vi "CE - PSD Marker Type.vi"(8 "error in (no error)":errorcluster, 11 "SA Measurement in":refnum<class "SA Measurement.lvclass">) -> (0 "error out":errorcluster, 3 "SA Measurement out":refnum<class "SA Measurement.lvclass">)   [LabVIEW 2023, in "Spectrum Analyzer.lvlib" / "SA Measurement.lvclass"]
uses:
  SA Measurement.lvclass
  SA Measurement.lvclass/SA Measurement.ctl
  Keysight 9020A/Keysight 9020A.lvclass
  TYPE DEFINITION/TYPE Y-axis Unit.ctl
  Spectrum Analyzer.lvlib
  TYPE DEFINITION/TYPE Start and Stop Frequency.ctl
  TYPE DEFINITION/TYPE Center and Span Frequency.ctl
  TYPE DEFINITION/TYPE Reference Level and Atten Param.ctl
  TYPE DEFINITION/TYPE Display Trace Mode Select.ctl
  TYPE DEFINITION/TYPE Detect Mode Select.ctl
  TYPE DEFINITION/TYPE Average Mode Select.ctl
  TYPE DEFINITION/SA Measurement Class/TYPE CE PSD Setting Parameter.ctl
  D:/Project/IST013_CE Conduction Measurement/IST013-CE-Condcuted-Measurement/src/Spectrum Analyzer/Interface_Spectrum/Interface_Spectrum.lvclass
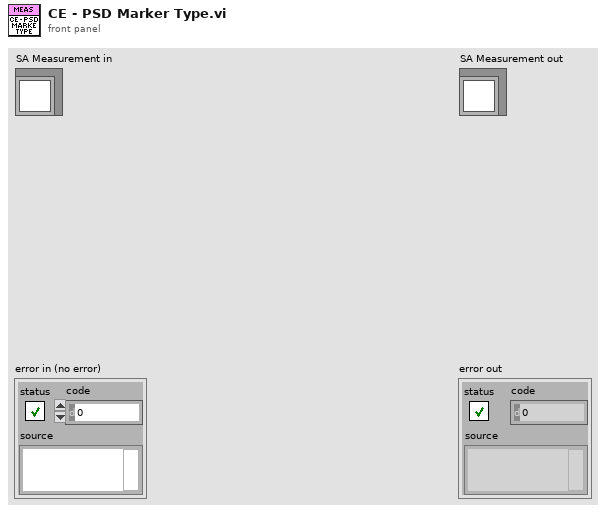
[diagram p1: front panel]
types:
  T1 = typedef "Spectrum Analyzer.lvlib/TYPE CE PSD Setting Parameter.ctl" = cluster{"Y-axis Unit":T2, "Start/Stop Frequency(Hz)":T3, "Center and Span Frequency(Hz)":T4, "PSD Type":enum16{"Marker", "Trace"}, "Ref and Atten":T5, "External Loss":dbl, "RBW/VBW(Hz)":cluster{"RBW":dbl, "VBW":dbl}, "Sweep Point":u32, "Sweep Time(s)":cluster{"Time":dbl, "Auto?":bool}, "Trace and Detect":cluster{"Trace Mode":T6, "Detector Type":T7, "Detect Auto?":bool}[], "Average Mode":T8, "Avg/Hold Number":u32}
  T2 = typedef "Spectrum Analyzer.lvlib/TYPE Y-axis Unit.ctl" = enum16{"dBm", "dBmV", "dBuV", "dBpW", "Volt", "Ampere", "Watt"}
  T3 = typedef "Spectrum Analyzer.lvlib/TYPE Start and Stop Frequency.ctl" = cluster{"Start":dbl, "Stop":dbl}
  T4 = typedef "Spectrum Analyzer.lvlib/TYPE Center and Span Frequency.ctl" = cluster{"Center":dbl, "Span":dbl}
  T5 = typedef "Spectrum Analyzer.lvlib/TYPE Reference Level and Atten Param.ctl" = cluster{"Reference Level":dbl, "Atten":i32, "Atten Auto?":bool, "Reference Level Offset":dbl}
  T6 = typedef "Spectrum Analyzer.lvlib/TYPE Display Trace Mode Select.ctl" = enum16{"Clear Write", "Max Hold", "Min Hold", "Average", "View"}
  T7 = typedef "Spectrum Analyzer.lvlib/TYPE Detect Mode Select.ctl" = enum16{"Det Auto (Normal)", "Auto Peak", "Positive Peak", "Negative Peak", "Sample", "RMS", "Average", "Quasipeak", "CISPR Average", "RMS Average"}
  T8 = typedef "Spectrum Analyzer.lvlib/TYPE Average Mode Select.ctl" = enum16{"Linear(Voltage Avg)", "Video(Log)", "Power"}
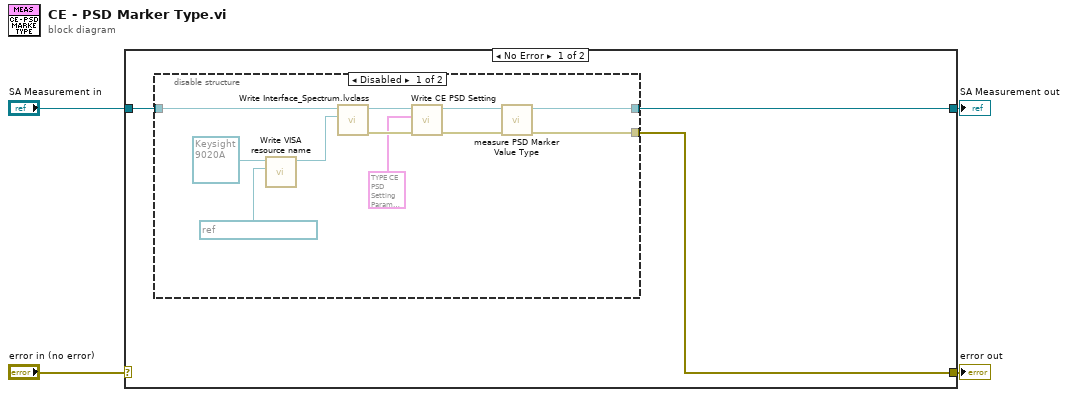
[diagram p0: block diagram]
diagram:
  n1 = case shown="No Error" "error in (no error)" {
    selector: "error in (no error)" -> [_ w20]
    tunnel: [w5 w20] -> w3
    tunnel: [w6 w19] -> w1
    tunnel: "SA Measurement in" -> [w7 w19]
    frame No Error {
      n2 = disable-structure shown="Disabled" {
        disable-tunnel: w7 -> [w16 _]
        disable-tunnel: [w10 _] -> w6
        disable-tunnel: [w8 _] -> w5
        frame Disabled {
          n3 = call "Write VISA resource name.vi"("VISA resource name"=refnum<visa-resource-name> "GPIB0::18::INSTR", "Keysight 9020A in"=refnum<class "Keysight 9020A.lvclass"> refnum ("Spectrum Analyzer.lvlib:Keysight 9020A.lvclass")) -> ("Keysight 9020A out"=w15:refnum<class "Keysight 9020A.lvclass">)  [unwired: 8 in, 1 out]
          n4 = call "Write Interface_Spectrum.lvclass.vi"("Interface_Spectrum.lvclass"=w15, "SA Measurement in"=w16) -> ("error out"=w13:errorcluster, "SA Measurement out"=w14:refnum<class "SA Measurement.lvclass">)  [unwired: 8 in]
          n5 = call "Write CE PSD Setting.vi"("error in (no error)"=w13, "CE PSD Setting"=T1 {"Y-axis Unit"=enum."dBm", "Start/Stop Frequency(Hz)"={"Start"=0.0, "Stop"=0.0}, "Center and Span Frequency(Hz)"={"Center"=2412000000.0, "Span"=20000000.0}, "PSD Type"=enum."Marker", "Ref and Atten"={"Reference Level"=0.0, "Atten"=20, "Atten Auto?"=FALSE, "Reference Level Offset"=0.0}, "External Loss"=10.0, "RBW/VBW(Hz)"={"RBW"=1000000.0, "VBW"=3000000.0}, "Sweep Point"=1001, "Sweep Time(s)"={"Time"=60.0, "Auto?"=FALSE}, "Trace and Detect"=[{"Trace Mode"=enum."Max Hold", "Detector Type"=enum."Average", "Detect Auto?"=FALSE}], "Average Mode"=enum."Power", "Avg/Hold Number"=1}, "SA Measurement in"=w14) -> ("error out"=w9:errorcluster, "SA Measurement out"=w11:refnum<class "SA Measurement.lvclass">)  [unwired: 7 in]
          n6 = call "measure PSD Marker Value Type.vi"("error in (no error)"=w9, "SA Measurement in"=w11) -> ("error out"=w8:errorcluster, "SA Measurement out"=w10:refnum<class "SA Measurement.lvclass">)  [unwired: 8 in]
        }
        frame Enabled {
        }
      }
    }
    frame Error {
    }
  }
  "error out" <- w3
  "SA Measurement out" <- w1
